vi "SPARK Get Absolute Encoder Config.vi"   [LabVIEW 2027]
doc: "Get the configuration of an absolute encoder connected to the data port of the SPARK."
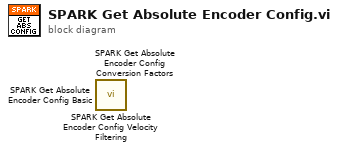
[diagram p0: block diagram]
diagram:
  n1 = call <vilib>:"SPARK Get Absolute Encoder Config Velocity Filtering.vi"() -> ()  [unwired: 9 in, 3 out]
  n2 = call <vilib>:"SPARK Get Absolute Encoder Config Conversion Factors.vi"() -> ()  [unwired: 8 in, 4 out]
  n3 = call <vilib>:"SPARK Get Absolute Encoder Config Basic.vi"() -> ()  [unwired: 7 in, 5 out]
